vi "Update Test-Assertion KVP.vi"(8 "error in (no error)":errorcluster, 10 "KVP":refnum<class "TestManagerMsg.KVP.lvclass">, 11 "Test Event Storage in":refnum<class "Test Event Storage.lvclass">) -> (0 "error out":errorcluster, 3 "Test Event Storage out":refnum<class "Test Event Storage.lvclass">)   [LabVIEW 2020, in "Caraya.lvlib" / "Test Event Storage.lvclass"]
uses:
  Test Event Storage.lvclass
  Test Manager Message KVP/TestManagerMsg.KVP.lvclass
  C:/projects/caraya/src/classes/Test Manager Message/TestManagerMsg.lvclass
  Test Event Storage.lvclass/Test Event Storage.ctl
  assert store -- cluster.ctl
  Test Manager Message Assertion/TestManagerMsg.Assertion.lvclass
  Test Manager Message Verbose/TestManagerMsg.Verbose.lvclass
  Test Manager Message/TestManagerMsg.lvclass/TestManagerMsg.ctl
  test store -- cluster.ctl
  Test Manager Message Test/TestManagerMsg.Test.lvclass
  Test Manager Message/TestManagerMsg.lvclass
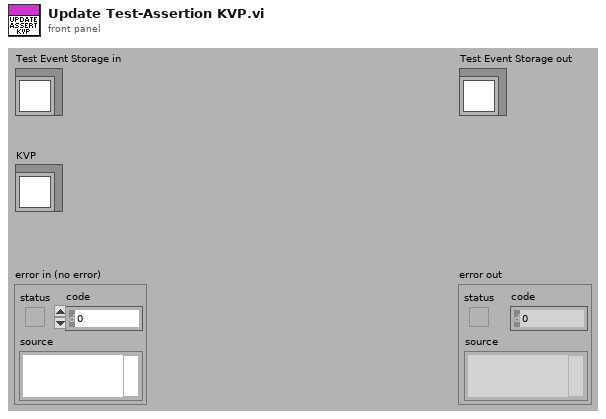
[diagram p1: front panel]
types:
  T1 = typedef "Caraya.lvlib/Test Event Storage.lvclass/assert store -- cluster.ctl" = cluster{"Assertion":refnum<class "TestManagerMsg.Assertion.lvclass">, "Explanation":refnum<class "TestManagerMsg.Verbose.lvclass">, "properties":variant, "measurements":variant, "user-defined":variant}
  T2 = typedef "Caraya.lvlib/Test Event Storage.lvclass/test store -- cluster.ctl" = cluster{"Test":refnum<class "TestManagerMsg.Test.lvclass">, "Defined":bool, "Passed":bool, "properties":variant, "assert-ids":variant}
  T3 = typedef "Caraya.lvlib/Test Event Storage.lvclass/Store Type -- enum.ctl" = enum16{"Suite", "Test", "Assert", "none"}
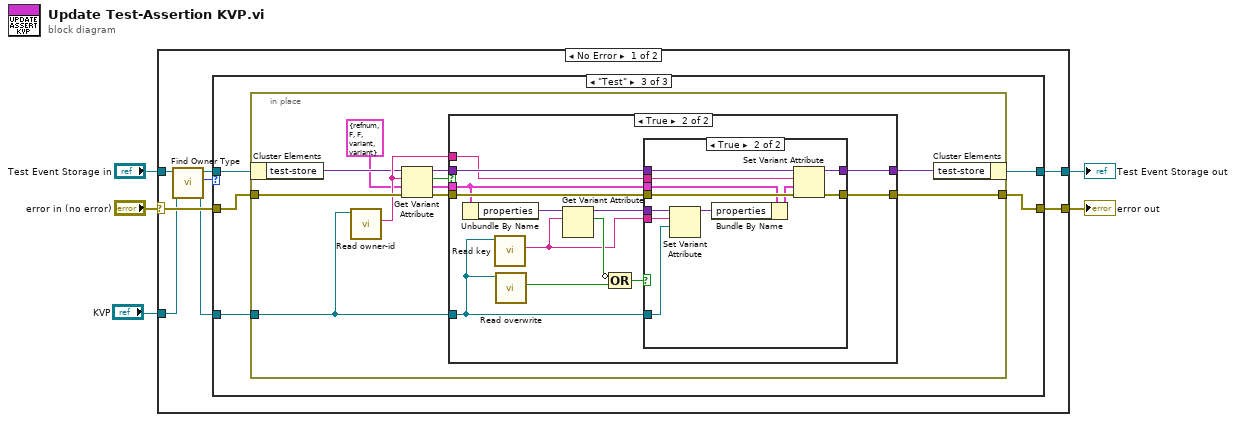
[diagram p0: block diagram]
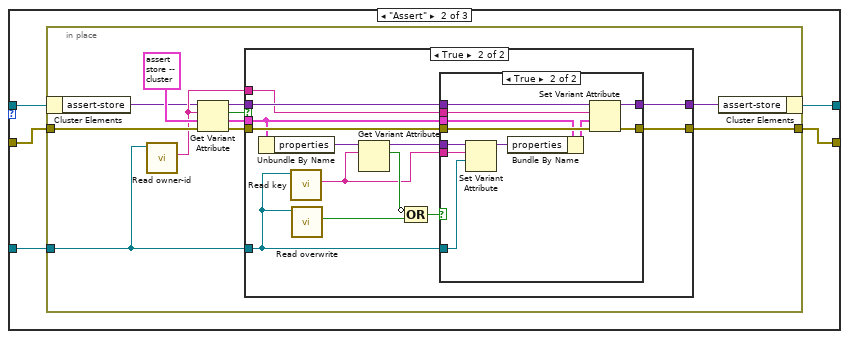
[diagram p3: hidden frame]
diagram:
  n1 = case shown="No Error" "error in (no error)" {
    selector: "error in (no error)" -> [w11 w105]
    tunnel: [w13 w105] -> w4
    tunnel: [w12 w104] -> w2
    tunnel: "Test Event Storage in" -> [w10 w104]
    tunnel: "KVP" -> [w7 _]
    frame No Error {
      n2 = call "Find Owner Type.vi"("Message"=w7, "Test Event Storage in"=w10) -> ("Message dup"=w6:refnum<class "TestManagerMsg.KVP.lvclass">, "Owner Type"=w8:T3, "Test Event Storage out"=w9:refnum<class "Test Event Storage.lvclass">)  [unwired: 7 in]
      n3 = case shown="\"Test\"" w8 {
        tunnel: w6 -> [_ w20 w64]
        tunnel: w11 -> [w14 w19 w63]
        tunnel: [w14 w18 w62] -> w13
        tunnel: [w15 w17 w61] -> w12
        tunnel: w9 -> [w15 w16 w60]
        frame "Suite", "none" {
          # "Not supported for Suites yet."
        }
        frame "Assert" {
          n4 = in-place {
            in-place-border: w19 -> [w29]
            in-place-border: [w30] -> w18
            in-place-border: w20 -> [w28]
            n5 = in-place-cluster #1(w16) -> ("assert-store"=w21:variant)
            n6 = call "Read owner-id.vi"("TestManagerMsg in"=w28) -> ("owner-id"=w22:string)  [unwired: 9 in, 1 out]
            n7 = Get Variant Attribute(Variant=w21, name=w22, default value (empty Variant)=T1 {"Assertion"=refnum, "Explanation"=refnum, "properties"=variant, "measurements"=variant, "user-defined"=variant} ("assert-store"), error in=w29) -> (duplicate Variant=w27:variant, found=w26:bool, value=w25:T1, error out=w24:errorcluster)
            n8 = case shown="True" w26 {
              tunnel: [w33 w46] -> w31
              tunnel: [w32 w45] -> w30
              tunnel: w24 -> [w32 w44]
              tunnel: w27 -> [w33 w43]
              tunnel: w22 -> [_ w42]
              tunnel: w25 -> [_ w41]
              tunnel: w28 -> [_ w38]
              frame False {
              }
              frame True {
                n9 = Unbundle By Name(w41) -> ("properties"=w39:variant)
                n10 = call "Read key.vi"("TestManagerMsg in"=w38) -> ("key"=w34:string)  [unwired: 9 in, 1 out]
                n11 = call "Read overwrite.vi"("TestManagerMsg in"=w38) -> ("overwrite?"=w36:bool)  [unwired: 9 in, 1 out]
                n12 = Get Variant Attribute(Variant=w39, name=w34) -> (duplicate Variant=w35:variant, found=w37:bool)  [unwired: 2 in, 2 out]
                n13 = Compound Arithmetic op=OR(invert w37, w36) -> (w40:bool)
                n14 = case shown="True" w40 {
                  tunnel: [w48 w59] -> w46
                  tunnel: [w47 w58] -> w45
                  tunnel: w44 -> [w47 w57]
                  tunnel: w43 -> [w48 w56]
                  tunnel: w42 -> [_ w55]
                  tunnel: w41 -> [_ w54]
                  tunnel: w38 -> [_ w49]
                  tunnel: w35 -> [_ w51]
                  tunnel: w34 -> [_ w50]
                  frame False {
                  }
                  frame True {
                    n15 = Set Variant Attribute(Variant=w51, name=w50, value=w49) -> (Variant out=w52:variant)  [unwired: 1 in, 2 out]
                    n16 = Bundle By Name(cluster=w54, "properties"=w52) -> (w53:T1)
                    n17 = Set Variant Attribute(Variant=w56, name=w55, value=w53, error in=w57) -> (Variant out=w59:variant, error out=w58:errorcluster)  [unwired: 1 out]
                  }
                }
              }
            }
            n18 = in-place-cluster #1("assert-store"=w31) -> (w17:refnum<class "Test Event Storage.lvclass">)
          }
        }
        frame "Test" {
          n19 = in-place {
            in-place-border: w63 -> [w73]
            in-place-border: [w74] -> w62
            in-place-border: w64 -> [w72]
            n20 = in-place-cluster #2(w60) -> ("test-store"=w66:variant)
            n21 = call "Read owner-id.vi"("TestManagerMsg in"=w72) -> ("owner-id"=w67:string)  [unwired: 9 in, 1 out]
            n22 = Get Variant Attribute(Variant=w66, name=w67, default value (empty Variant)=T2 {"Test"=refnum, "Defined"=FALSE, "Passed"=FALSE, "properties"=variant, "assert-ids"=variant} ("test-store"), error in=w73) -> (duplicate Variant=w71:variant, found=w70:bool, value=w69:T2, error out=w68:errorcluster)
            n23 = case shown="True" w70 {
              tunnel: [w77 w90] -> w75
              tunnel: [w76 w89] -> w74
              tunnel: w68 -> [w76 w88]
              tunnel: w71 -> [w77 w87]
              tunnel: w67 -> [_ w86]
              tunnel: w69 -> [_ w85]
              tunnel: w72 -> [_ w82]
              frame False {
              }
              frame True {
                n24 = Unbundle By Name(w85) -> ("properties"=w83:variant)
                n25 = call "Read key.vi"("TestManagerMsg in"=w82) -> ("key"=w78:string)  [unwired: 9 in, 1 out]
                n26 = call "Read overwrite.vi"("TestManagerMsg in"=w82) -> ("overwrite?"=w80:bool)  [unwired: 9 in, 1 out]
                n27 = Get Variant Attribute(Variant=w83, name=w78) -> (duplicate Variant=w79:variant, found=w81:bool)  [unwired: 2 in, 2 out]
                n28 = Compound Arithmetic op=OR(invert w81, w80) -> (w84:bool)
                n29 = case shown="True" w84 {
                  tunnel: [w92 w103] -> w90
                  tunnel: [w91 w102] -> w89
                  tunnel: w88 -> [w91 w101]
                  tunnel: w87 -> [w92 w100]
                  tunnel: w86 -> [_ w99]
                  tunnel: w85 -> [_ w98]
                  tunnel: w82 -> [_ w93]
                  tunnel: w79 -> [_ w95]
                  tunnel: w78 -> [_ w94]
                  frame False {
                  }
                  frame True {
                    n30 = Set Variant Attribute(Variant=w95, name=w94, value=w93) -> (Variant out=w96:variant)  [unwired: 1 in, 2 out]
                    n31 = Bundle By Name(cluster=w98, "properties"=w96) -> (w97:T2)
                    n32 = Set Variant Attribute(Variant=w100, name=w99, value=w97, error in=w101) -> (Variant out=w103:variant, error out=w102:errorcluster)  [unwired: 1 out]
                  }
                }
              }
            }
            n33 = in-place-cluster #2("test-store"=w75) -> (w61:refnum<class "Test Event Storage.lvclass">)
          }
        }
      }
    }
    frame Error {
    }
  }
  "error out" <- w4
  "Test Event Storage out" <- w2
